vi "Comparaison_profils EPC3000.vi"(3 "Configs + progs régulateurs":T1(array[cluster])) -> (0 "Profils":T2(array[cluster]))   [LabVIEW 2022 SP3]
uses:
  Variables globales/Variables glob EUROTHERM.vi
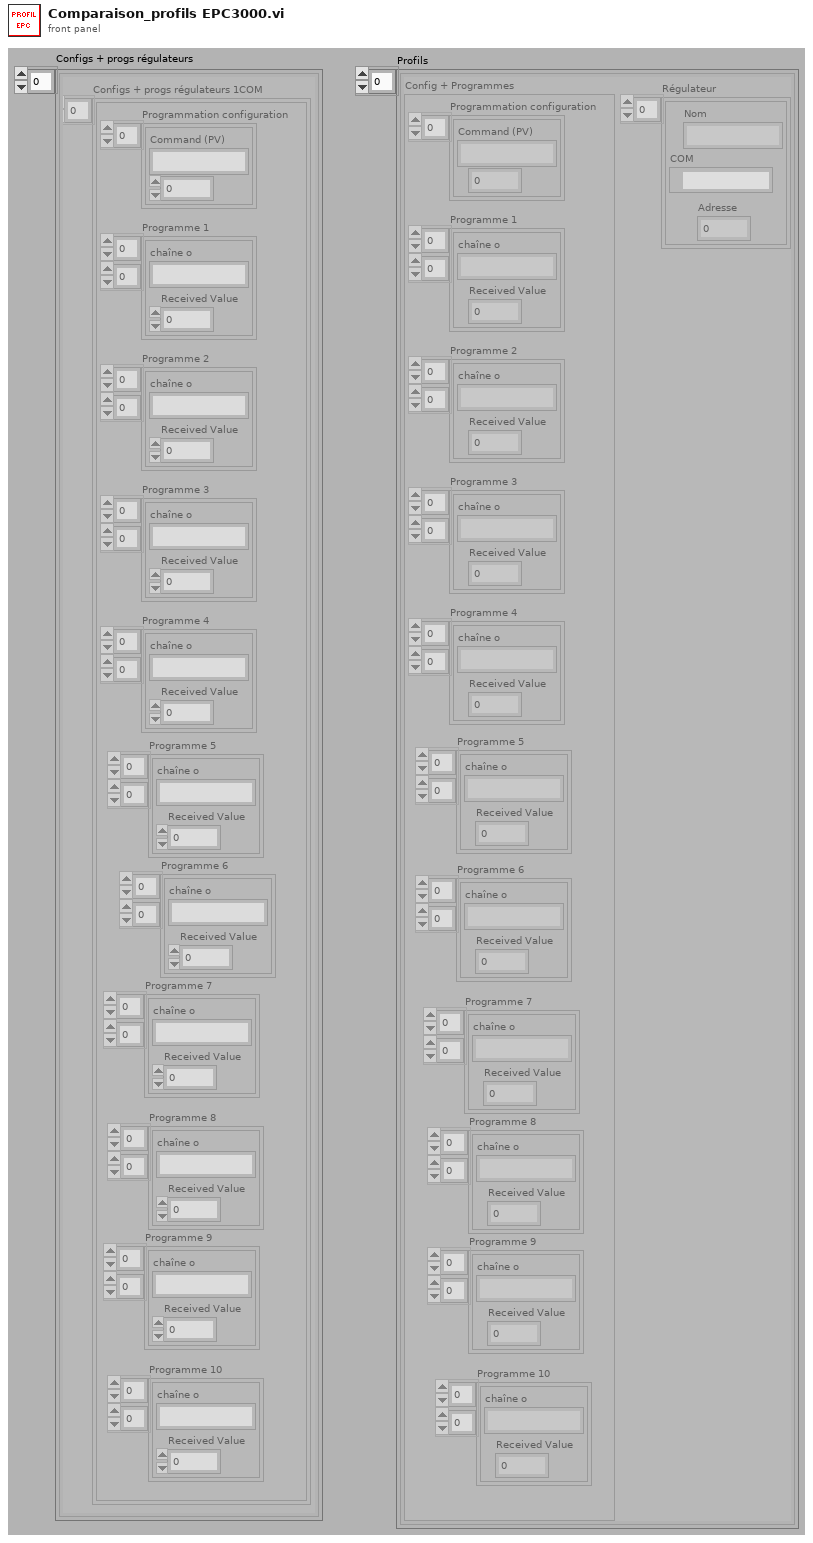
[diagram p1: front panel]
types:
  T1 = cluster{"Configs + progs régulateurs 1COM":cluster{"Programmation configuration":cluster{"Command (PV)":string, dbl}[], "Programme 1":cluster{"chaîne o":string, "Received Value":dbl}[][], "Programme 2":cluster{"chaîne o":string, "Received Value":dbl}[][], "Programme 3":cluster{"chaîne o":string, "Received Value":dbl}[][], "Programme 4":cluster{"chaîne o":string, "Received Value":dbl}[][], "Programme 5":cluster{"chaîne o":string, "Received Value":dbl}[][], "Programme 6":cluster{"chaîne o":string, "Received Value":dbl}[][], "Programme 7":cluster{"chaîne o":string, "Received Value":dbl}[][], "Programme 8":cluster{"chaîne o":string, "Received Value":dbl}[][], "Programme 9":cluster{"chaîne o":string, "Received Value":dbl}[][], "Programme 10":cluster{"chaîne o":string, "Received Value":dbl}[][]}[]}[]
  T2 = cluster{"Config + Programmes":cluster{"Programmation configuration":cluster{"Command (PV)":string, dbl}[], "Programme 1":cluster{"chaîne o":string, "Received Value":dbl}[][], "Programme 2":cluster{"chaîne o":string, "Received Value":dbl}[][], "Programme 3":cluster{"chaîne o":string, "Received Value":dbl}[][], "Programme 4":cluster{"chaîne o":string, "Received Value":dbl}[][], "Programme 5":cluster{"chaîne o":string, "Received Value":dbl}[][], "Programme 6":cluster{"chaîne o":string, "Received Value":dbl}[][], "Programme 7":cluster{"chaîne o":string, "Received Value":dbl}[][], "Programme 8":cluster{"chaîne o":string, "Received Value":dbl}[][], "Programme 9":cluster{"chaîne o":string, "Received Value":dbl}[][], "Programme 10":cluster{"chaîne o":string, "Received Value":dbl}[][]}, "Régulateur":cluster{"Nom":string, "COM":refnum<visa-resource-name>, "Adresse":u8}[]}[]
  T3 = cluster{"Nom":string, "COM":refnum<visa-resource-name>, "Adresse":u8}
  T4 = cluster{cluster{"Nom":string, "COM":refnum<visa-resource-name>, "Adresse":u8}[]}
  T5 = cluster{"Configs + progs régulateurs 1COM":cluster{"Programmation configuration":cluster{"Command (PV)":string, dbl}[], "Programme 1":cluster{"chaîne o":string, "Received Value":dbl}[][], "Programme 2":cluster{"chaîne o":string, "Received Value":dbl}[][], "Programme 3":cluster{"chaîne o":string, "Received Value":dbl}[][], "Programme 4":cluster{"chaîne o":string, "Received Value":dbl}[][], "Programme 5":cluster{"chaîne o":string, "Received Value":dbl}[][], "Programme 6":cluster{"chaîne o":string, "Received Value":dbl}[][], "Programme 7":cluster{"chaîne o":string, "Received Value":dbl}[][], "Programme 8":cluster{"chaîne o":string, "Received Value":dbl}[][], "Programme 9":cluster{"chaîne o":string, "Received Value":dbl}[][], "Programme 10":cluster{"chaîne o":string, "Received Value":dbl}[][]}[]}
  T6 = cluster{"Nom":string, "COM":refnum<visa-resource-name>, "Adresse":u8}[]
  T7 = cluster{"Programmation configuration":cluster{"Command (PV)":string, dbl}[], "Programme 1":cluster{"chaîne o":string, "Received Value":dbl}[][], "Programme 2":cluster{"chaîne o":string, "Received Value":dbl}[][], "Programme 3":cluster{"chaîne o":string, "Received Value":dbl}[][], "Programme 4":cluster{"chaîne o":string, "Received Value":dbl}[][], "Programme 5":cluster{"chaîne o":string, "Received Value":dbl}[][], "Programme 6":cluster{"chaîne o":string, "Received Value":dbl}[][], "Programme 7":cluster{"chaîne o":string, "Received Value":dbl}[][], "Programme 8":cluster{"chaîne o":string, "Received Value":dbl}[][], "Programme 9":cluster{"chaîne o":string, "Received Value":dbl}[][], "Programme 10":cluster{"chaîne o":string, "Received Value":dbl}[][]}[]
  T8 = cluster{"Programmation configuration":cluster{"Command (PV)":string, dbl}[], "Programme 1":cluster{"chaîne o":string, "Received Value":dbl}[][], "Programme 2":cluster{"chaîne o":string, "Received Value":dbl}[][], "Programme 3":cluster{"chaîne o":string, "Received Value":dbl}[][], "Programme 4":cluster{"chaîne o":string, "Received Value":dbl}[][], "Programme 5":cluster{"chaîne o":string, "Received Value":dbl}[][], "Programme 6":cluster{"chaîne o":string, "Received Value":dbl}[][], "Programme 7":cluster{"chaîne o":string, "Received Value":dbl}[][], "Programme 8":cluster{"chaîne o":string, "Received Value":dbl}[][], "Programme 9":cluster{"chaîne o":string, "Received Value":dbl}[][], "Programme 10":cluster{"chaîne o":string, "Received Value":dbl}[][]}
  T9 = cluster{"Config + Programmes":cluster{"Programmation configuration":cluster{"Command (PV)":string, dbl}[], "Programme 1":cluster{"chaîne o":string, "Received Value":dbl}[][], "Programme 2":cluster{"chaîne o":string, "Received Value":dbl}[][], "Programme 3":cluster{"chaîne o":string, "Received Value":dbl}[][], "Programme 4":cluster{"chaîne o":string, "Received Value":dbl}[][], "Programme 5":cluster{"chaîne o":string, "Received Value":dbl}[][], "Programme 6":cluster{"chaîne o":string, "Received Value":dbl}[][], "Programme 7":cluster{"chaîne o":string, "Received Value":dbl}[][], "Programme 8":cluster{"chaîne o":string, "Received Value":dbl}[][], "Programme 9":cluster{"chaîne o":string, "Received Value":dbl}[][], "Programme 10":cluster{"chaîne o":string, "Received Value":dbl}[][]}, cluster{"Nom":string, "COM":refnum<visa-resource-name>, "Adresse":u8}[]}
  T10 = cluster{"Config + Programmes":cluster{"Programmation configuration":cluster{"Command (PV)":string, dbl}[], "Programme 1":cluster{"chaîne o":string, "Received Value":dbl}[][], "Programme 2":cluster{"chaîne o":string, "Received Value":dbl}[][], "Programme 3":cluster{"chaîne o":string, "Received Value":dbl}[][], "Programme 4":cluster{"chaîne o":string, "Received Value":dbl}[][], "Programme 5":cluster{"chaîne o":string, "Received Value":dbl}[][], "Programme 6":cluster{"chaîne o":string, "Received Value":dbl}[][], "Programme 7":cluster{"chaîne o":string, "Received Value":dbl}[][], "Programme 8":cluster{"chaîne o":string, "Received Value":dbl}[][], "Programme 9":cluster{"chaîne o":string, "Received Value":dbl}[][], "Programme 10":cluster{"chaîne o":string, "Received Value":dbl}[][]}, cluster{"Nom":string, "COM":refnum<visa-resource-name>, "Adresse":u8}[]}[]
  T11 = cluster{"Programmation configuration":cluster{"Command (PV)":bool, bool}[], "Programme 1":cluster{"chaîne o":bool, "Received Value":bool}[][], "Programme 2":cluster{"chaîne o":bool, "Received Value":bool}[][], "Programme 3":cluster{"chaîne o":bool, "Received Value":bool}[][], "Programme 4":cluster{"chaîne o":bool, "Received Value":bool}[][], "Programme 5":cluster{"chaîne o":bool, "Received Value":bool}[][], "Programme 6":cluster{"chaîne o":bool, "Received Value":bool}[][], "Programme 7":cluster{"chaîne o":bool, "Received Value":bool}[][], "Programme 8":cluster{"chaîne o":bool, "Received Value":bool}[][], "Programme 9":cluster{"chaîne o":bool, "Received Value":bool}[][], "Programme 10":cluster{"chaîne o":bool, "Received Value":bool}[][]}
  T12 = cluster{"chaîne o":bool, "Received Value":bool}[][]
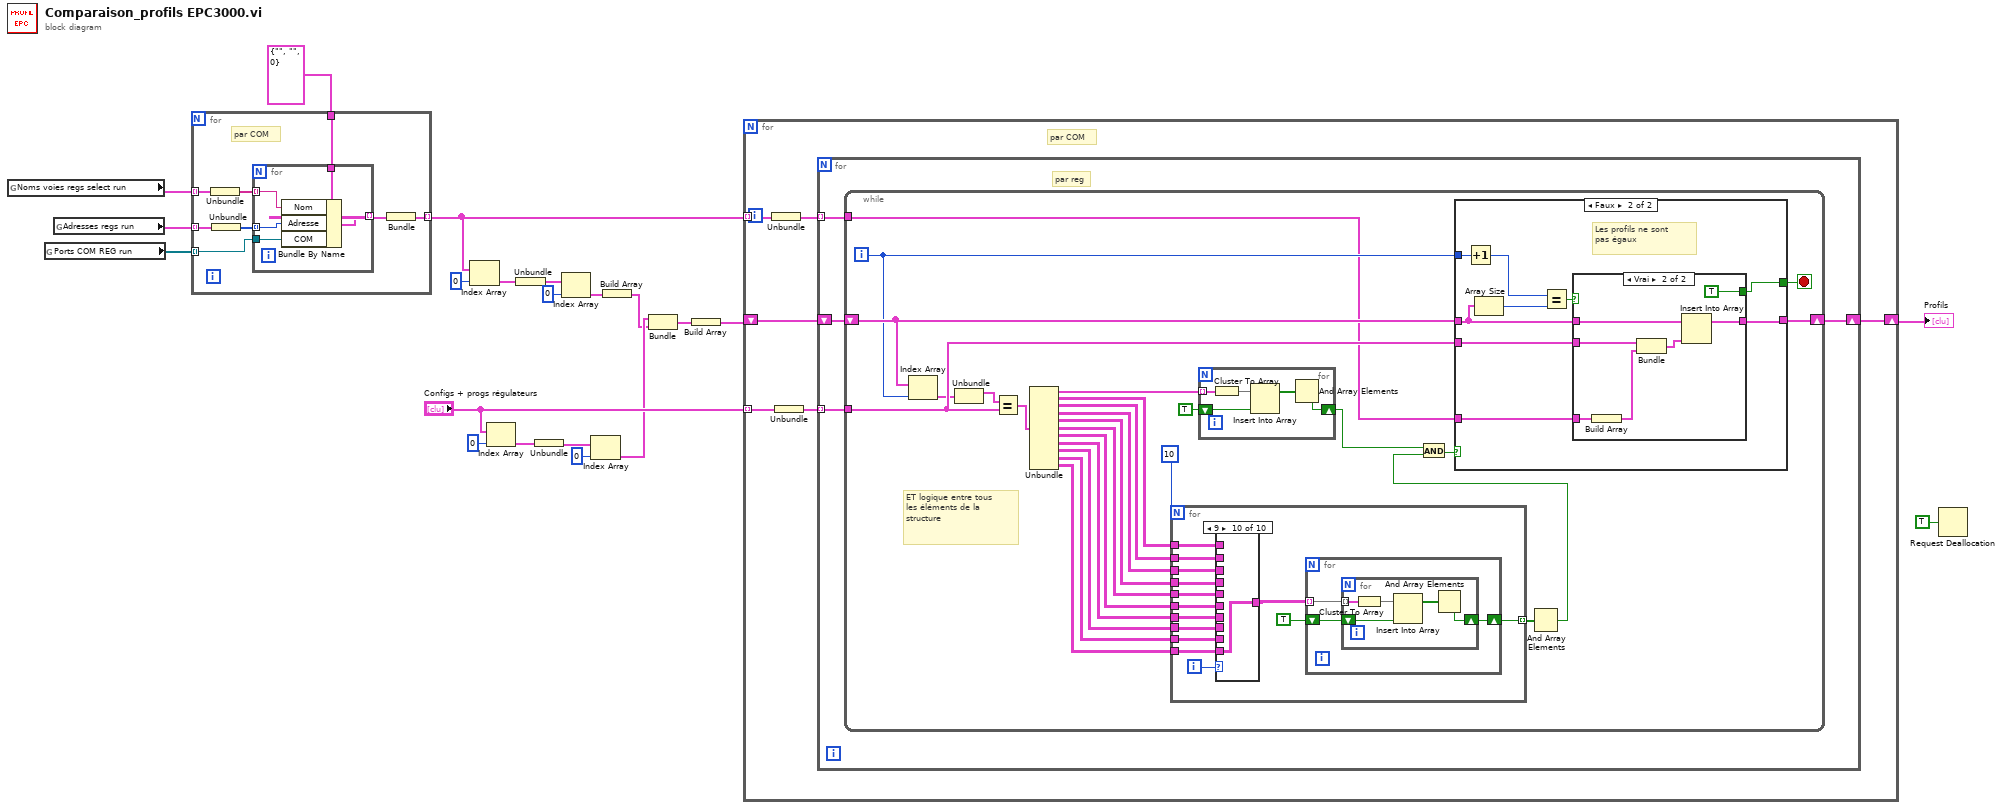
[diagram p0: block diagram]
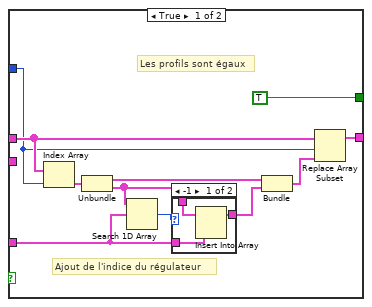
[diagram p11: hidden frame]
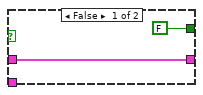
[diagram p13: hidden frame]
diagram:
  n1 = global read "Variables glob EUROTHERM.vi" "Noms voies regs select run"() -> (w18:cluster{"Noms voies select run 1COM":string[]}[])
  n2 = global read "Variables glob EUROTHERM.vi" "Ports COM REG run"() -> (w1:refnum<visa-resource-name>[])
  n3 = global read "Variables glob EUROTHERM.vi" "Adresses regs run"() -> (w19:cluster{"Adresses run 1COM reg":u16[]}[])
  n4 = for {
    tunnel: w18 -> [w27] mode=indexing
    tunnel: w19 -> [w29] mode=indexing
    tunnel: [w24] -> w12 mode=indexing
    tunnel: w1 -> [w22] mode=indexing
    tunnel: T3 {"Nom"="", "COM"="", "Adresse"=0} -> [w23]
    # "par COM"
    n5 = Unbundle(w27) -> ("Noms voies select run 1COM"=w26:string[])
    n6 = Unbundle(w29) -> ("Adresses run 1COM reg"=w28:u16[])
    n7 = for {
      tunnel: w26 -> [w30] mode=indexing
      tunnel: w28 -> [w31] mode=indexing
      tunnel: [w34] -> w25 mode=indexing
      tunnel: w23 -> [w33]
      tunnel: w22 -> [w32]
      n8 = Bundle By Name(cluster=w33, "Nom"=w30, "Adresse"=w31, "COM"=w32) -> (w34:T3)
    }
    n9 = Bundle(w25) -> (w24:T4)  [unwired: 1 in]
  }
  n10 = Index Array(array=w12, index=0 ("indice")) -> (element=w10:T4)
  n11 = Index Array(array="Configs + progs régulateurs", index=0 ("indice")) -> (element=w15:T5)
  n12 = Unbundle(w10) -> (w9:T6)
  n13 = Unbundle(w15) -> ("Configs + progs régulateurs 1COM"=w14:T7)
  n14 = Index Array(array=w9, index=0 ("indice")) -> (element=w7:T3)
  n15 = Index Array(array=w14, index=0 ("indice")) -> (element=w6:T8)
  n16 = Build Array(w7) -> (w5:T6)
  n17 = Bundle("Config + Programmes"=w6, w5) -> (w4:T9)  [unwired: 1 in]
  n18 = Build Array(w4) -> (w3:T10)
  n19 = for {
    shift-right: [w39] -> w21
    shift-left: w3 -> [w40]
    tunnel: "Configs + progs régulateurs" -> [w38] mode=indexing
    tunnel: w12 -> [w36] mode=indexing
    # "par COM"
    n20 = Unbundle(w36) -> (w35:T6)
    n21 = Unbundle(w38) -> ("Configs + progs régulateurs 1COM"=w37:T7)
    n22 = for {
      tunnel: w37 -> [w43] mode=indexing
      tunnel: w35 -> [w42] mode=indexing
      shift-right: [w41] -> w39
      shift-left: w40 -> [w44]
      # "par reg"
      n23 = while {
        tunnel: w43 -> [w67]
        shift-right: [w65] -> w41
        shift-left: w44 -> [w64]
        tunnel: w42 -> [w61]
        i -> [w63]
        stop <- w62 stop-if-true
        # "ET logique entre tous les éléments de la structure"
        n24 = Index Array(array=w64, index=w63) -> (element=w66:T9)
        n25 = Unbundle(w66) -> ("Config + Programmes"=w68:T8)  [unwired: 1 out]
        n26 = Equal?(x=w68, y=w67) -> (x = y?=w57:T11)
        n27 = Unbundle(w57) -> ("Programmation configuration"=w70:cluster{"Command (PV)":bool, bool}[], "Programme 1"=w46:T12, "Programme 2"=w47:T12, "Programme 3"=w48:T12, "Programme 4"=w49:T12, "Programme 5"=w50:T12, "Programme 6"=w51:T12, "Programme 7"=w52:T12, "Programme 8"=w53:T12, "Programme 9"=w54:T12, "Programme 10"=w55:T12)
        n28 = for {
          N: 10 -> [_]
          tunnel: w55 -> [w74]
          tunnel: w54 -> [w75]
          tunnel: w53 -> [w76]
          tunnel: w52 -> [w77]
          tunnel: w51 -> [w78]
          tunnel: w50 -> [w79]
          tunnel: w49 -> [w80]
          tunnel: w48 -> [w81]
          tunnel: w47 -> [w82]
          tunnel: w46 -> [w83]
          tunnel: [w71] -> w45 mode=indexing
          i -> [w84]
          n29 = case shown="9" w84 {
            tunnel: w83 -> [w93 _ _ _ _ _ _ _ _ _]
            tunnel: w82 -> [_ w94 _ _ _ _ _ _ _ _]
            tunnel: w81 -> [_ _ w95 _ _ _ _ _ _ _]
            tunnel: w80 -> [_ _ _ w96 _ _ _ _ _ _]
            tunnel: w79 -> [_ _ _ _ w97 _ _ _ _ _]
            tunnel: w78 -> [_ _ _ _ _ w98 _ _ _ _]
            tunnel: w77 -> [_ _ _ _ _ _ w99 _ _ _]
            tunnel: w76 -> [_ _ _ _ _ _ _ w100 _ _]
            tunnel: w75 -> [_ _ _ _ _ _ _ _ w101 _]
            tunnel: w74 -> [_ _ _ _ _ _ _ _ _ w102]
            tunnel: [w93 w94 w95 w96 w97 w98 w99 w100 w101 w102] -> w72
            frame 0, Default {
            }
            frame 1 {
            }
            frame 2 {
            }
            frame 3 {
            }
            frame 4 {
            }
            frame 5 {
            }
            frame 6 {
            }
            frame 7 {
            }
            frame 8 {
            }
            frame 9 {
            }
          }
          n30 = for {
            tunnel: w72 -> [w87] mode=indexing
            shift-right: [w85] -> w71
            shift-left: TRUE -> [w86]
            n31 = for {
              tunnel: w87 -> [w92] mode=indexing
              shift-right: [w91] -> w85
              shift-left: w86 -> [w90]
              n32 = Cluster To Array(cluster=w92) -> (array=w89:bool[])
              n33 = Insert Into Array(array=w89, new element=w90) -> (w88:bool[])  [unwired: 1 in]
              n34 = And Array Elements(Boolean array=w88) -> (logical AND=w91:bool)
            }
          }
        }
        n35 = for {
          tunnel: w70 -> [w140] mode=indexing
          shift-right: [w139] -> w60
          shift-left: TRUE -> [w138]
          n36 = Cluster To Array(cluster=w140) -> (array=w137:bool[])
          n37 = Insert Into Array(array=w137, new element=w138) -> (w136:bool[])  [unwired: 1 in]
          n38 = And Array Elements(Boolean array=w136) -> (logical AND=w139:bool)
        }
        n39 = And Array Elements(Boolean array=w45) -> (logical AND=w59:bool)
        n40 = And(x=w60, y=w59) -> (x .and. y?=w58:bool)
        n41 = case shown="Faux" w58 {
          tunnel: [TRUE w119] -> w62
          tunnel: w67 -> [_ w126]
          tunnel: w64 -> [w109 w124]
          tunnel: w63 -> [w106 w123]
          tunnel: [w108 w125] -> w65
          tunnel: w61 -> [w104 w118]
          frame True {
            # "Ajout de l'indice du régulateur"
            # "Les profils sont égaux"
            n42 = Index Array(array=w109, index=w106) -> (element=w110:T9)
            n43 = Unbundle(w110) -> ("Config + Programmes"=w113:T8, w105:T6)
            n44 = Search 1D Array(1D array=w105, element=w104) -> (index of element=w103:i32)  [unwired: 1 in]
            n45 = case shown="-1" w103 {
              tunnel: [w116 w117] -> w112
              tunnel: w105 -> [w115 w117]
              tunnel: w104 -> [w114 _]
              frame -1 {
                n46 = Insert Into Array(array=w115, new element=w114) -> (w116:T6)  [unwired: 1 in]
              }
              frame 0, Default {
              }
            }
            n47 = Bundle("Config + Programmes"=w113, w112) -> (w107:T9)  [unwired: 1 in]
            n48 = Replace Array Subset(array=w109, new element=w107, index=w106) -> (w108:T10)
          }
          frame False {
            # "Les profils ne sont pas égaux"
            n49 = Increment(x=w123) -> (x+1=w121:i32)
            n50 = Array Size(array=w124) -> (size(s)=w122:i32)
            n51 = Equal?(x=w121, y=w122) -> (x = y?=w120:bool)
            n52 = case shown="Vrai" w120 {
              tunnel: w126 -> [_ w135]
              tunnel: [w128 w134] -> w125
              tunnel: w124 -> [w128 w133]
              tunnel: [FALSE TRUE] -> w119
              tunnel: w118 -> [_ w131]
              frame False {
              }
              frame True {
                n53 = Build Array(w131) -> (w130:T6)
                n54 = Bundle("Config + Programmes"=w135, w130) -> (w129:T9)  [unwired: 1 in]
                n55 = Insert Into Array(array=w133, new element=w129) -> (w134:T10)  [unwired: 1 in]
              }
            }
          }
        }
      }
    }
  }
  "Profils" <- w21
  n56 = Request Deallocation(TRUE ("flag")) -> ()
